vi "Test Format Entry Row.vi"(8 "error in":errorcluster, 10 "Work Folder":path, 11 "Test Data Folder":path) -> (0 "error out":errorcluster, 2 "Report":string, 3 "Passed":bool)   [LabVIEW 2026]
doc: "Tests Format Entry Row.vi with the Project Store of the schema-v2 sample data (Test Data\\Samples, copied into a new case folder). Checks: a row has the seven columns of the old TimeCard row (ID, Start, End, Elapsed, Project, Task, Description); an elapsed time of 59.6 s shows 00:01:00 and not 00:00:60; project and task names are looked up by ID; the Start column is the local time formatted %I:%M:%S %p; a running entry (End Time 0) gets an empty End column and an Elapsed of Now minus Start; an unknown Project ID is shown as the ID.\n\nInputs: Test Data Folder; Work Folder; error in. Outputs: Passed; Report; error out.\n\nGenerated by: Claude"
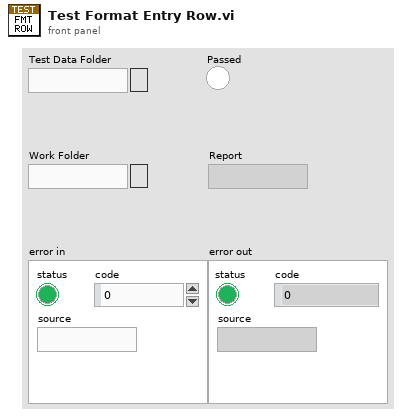
[diagram p1: front panel]
types:
  T1 = cluster{"ID":string, "Project ID":string, "Task ID":string, timestamp, timestamp, "Description":string}
  T2 = cluster{"ID":string, "Project ID":string, "Task ID":string, timestamp, "zero time":timestamp, "Description":string}
  T3 = cluster{"ID":string, "unknown project":string, "Task ID":string, timestamp, timestamp, "Description":string}
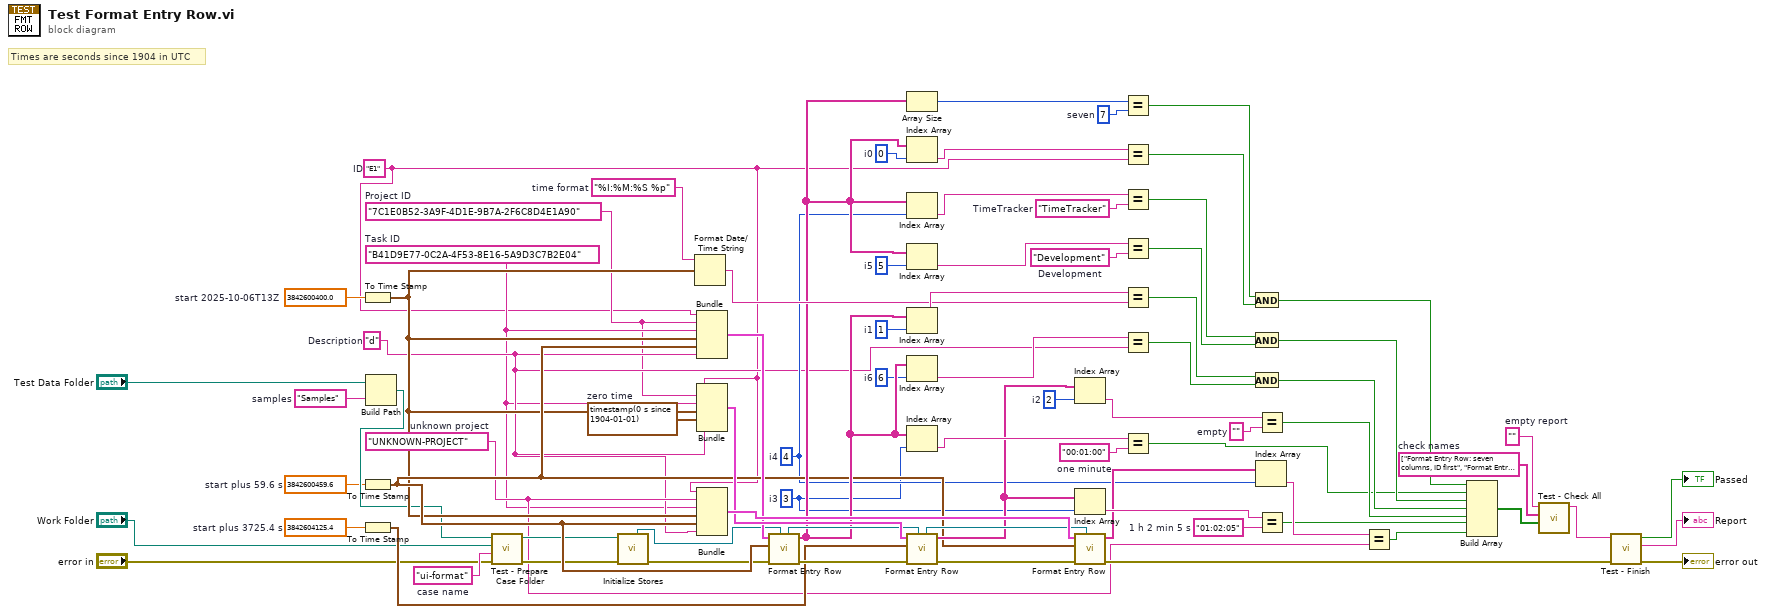
[diagram p0: block diagram]
diagram:
  w33 = string[] ["Format Entry Row: seven columns, ID first", "Format Entry Row: elapsed 59.6 s shows 00:01:00 (not 00:00:60)", "Format Entry Row: project and task names looked up by ID", "Format Entry Row: Start column is local %I:%M:%S %p and Description is last", "Format Entry Row: running entry leaves End empty", "Format Entry Row: running entry Elapsed is Now minus Start (01:02:05)", "Format Entry Row: unknown Project ID is shown as the ID"]  # check names
  w32 = "01:02:05"  # 1 h 2 min 5 s
  w31 = ""  # empty
  w30 = "Development"  # Development
  w29 = "TimeTracker"  # TimeTracker
  w28 = "00:01:00"  # one minute
  w27 = 6  # i6
  w26 = 5  # i5
  w25 = 4  # i4
  w24 = 3  # i3
  w23 = 2  # i2
  w22 = 1  # i1
  w21 = 0  # i0
  w20 = 7  # seven
  w19 = "%I:%M:%S %p"  # time format
  w18 = "UNKNOWN-PROJECT"  # unknown project
  w17 = timestamp(0 s since 1904-01-01)  # zero time
  w16 = 3842604125.4  # start plus 3725.4 s
  w15 = 3842600459.6  # start plus 59.6 s
  w14 = 3842600400.0  # start 2025-10-06T13Z
  w13 = "d"  # Description
  w12 = "B41D9E77-0C2A-4F53-8E16-5A9D3C7B2E04"  # Task ID
  w11 = "7C1E0B52-3A9F-4D1E-9B7A-2F6C8D4E1A90"  # Project ID
  w10 = "E1"  # ID
  w9 = ""  # empty report
  w8 = "ui-format"  # case name
  w7 = "Samples"  # samples
  # "Times are seconds since 1904 in UTC"
  n1 = To Time Stamp(1:w14) -> (0:w39:timestamp)
  n2 = To Time Stamp(1:w15) -> (0:w40:timestamp)
  n3 = To Time Stamp(1:w16) -> (0:w41:timestamp)
  n4 = Build Path(base path="Test Data Folder", name or relative path=w7) -> (appended path=w34:path)
  n5 = call "Test - Prepare Case Folder.vi"("error in (no error)"="error in", "Case Name"=w8, "Work Folder"="Work Folder", "Source Folder"=w34) -> ("error out"=w36:errorcluster, "Case Folder"=w35:path)  [unwired: 6 in]
  n6 = call "Initialize Stores.vi"("error in"=w36, "Data Folder"=w35) -> ("error out"=w38:errorcluster, "Project Store out"=w37:refnum<class "Project Store.lvclass">)  [unwired: 5 in, 3 out]
  n7 = Format Date/Time String(time format string (%c)=w19, seconds (now)=w39) -> (date/time string=w65:string)  [unwired: 1 out]
  n8 = Bundle("ID"=w10, "Project ID"=w11, "Task ID"=w12, w39, w40, "Description"=w13) -> (w42:T1)  [unwired: 1 in]
  n9 = Bundle("ID"=w10, "Project ID"=w11, "Task ID"=w12, w39, "zero time"=w17, "Description"=w13) -> (w46:T2)  [unwired: 1 in]
  n10 = Bundle("ID"=w10, "unknown project"=w18, "Task ID"=w12, w39, w40, "Description"=w13) -> (w50:T3)  [unwired: 1 in]
  n11 = call "Format Entry Row.vi"("Project Store in"=w37, "error in"=w38, "Now"=w40, "Time Entry"=w42) -> ("error out"=w45:errorcluster, "Row"=w43:string[], "Project Store out"=w44:refnum<class "Project Store.lvclass">)  [unwired: 5 in]
  n12 = Array Size(array=w43) -> (size(s)=w53:i32)
  n13 = Index Array(array=w43, index=w21) -> (element=w55:string)
  n14 = Index Array(array=w43, index=w25) -> (element=w60:string)
  n15 = Index Array(array=w43, index=w26) -> (element=w61:string)
  n16 = Index Array(array=w43, index=w22) -> (element=w66:string)
  n17 = Index Array(array=w43, index=w27) -> (element=w68:string)
  n18 = Index Array(array=w43, index=w24) -> (element=w58:string)
  n19 = call "Format Entry Row.vi"("Project Store in"=w44, "error in"=w45, "Now"=w41, "Time Entry"=w46) -> ("error out"=w49:errorcluster, "Row"=w47:string[], "Project Store out"=w48:refnum<class "Project Store.lvclass">)  [unwired: 5 in]
  n20 = Index Array(array=w47, index=w23) -> (element=w71:string)
  n21 = Index Array(array=w47, index=w24) -> (element=w73:string)
  n22 = call "Format Entry Row.vi"("Project Store in"=w48, "error in"=w49, "Now"=w40, "Time Entry"=w50) -> ("error out"=w52:errorcluster, "Row"=w51:string[])  [unwired: 5 in, 1 out]
  n23 = Equal?(x=w53, y=w20) -> (x = y?=w54:bool)
  n24 = Equal?(x=w55, y=w10) -> (x = y?=w56:bool)
  n25 = Equal?(x=w60, y=w29) -> (x = y?=w62:bool)
  n26 = Equal?(x=w61, y=w30) -> (x = y?=w63:bool)
  n27 = Equal?(x=w66, y=w65) -> (x = y?=w67:bool)
  n28 = Equal?(x=w68, y=w13) -> (x = y?=w69:bool)
  n29 = Equal?(x=w58, y=w28) -> (x = y?=w59:bool)
  n30 = And(x=w54, y=w56) -> (x .and. y?=w57:bool)
  n31 = And(x=w62, y=w63) -> (x .and. y?=w64:bool)
  n32 = And(x=w67, y=w69) -> (x .and. y?=w70:bool)
  n33 = Index Array(array=w51, index=w25) -> (element=w75:string)
  n34 = Equal?(x=w71, y=w31) -> (x = y?=w72:bool)
  n35 = Equal?(x=w73, y=w32) -> (x = y?=w74:bool)
  n36 = Equal?(x=w75, y=w18) -> (x = y?=w76:bool)
  n37 = Build Array(w57, w59, w64, w70, w72, w74, w76) -> (w77:bool[])
  n38 = call "Test - Check All.vi"("Conditions"=w77, "Check Names"=w33, "Report in"=w9) -> ("Report out"=w78:string)  [unwired: 7 in, 1 out]
  n39 = call "Test - Finish.vi"("error in (no error)"=w52, "Report"=w78) -> ("error out"=→"error out":errorcluster, "Report out"=→"Report":string, "Passed"=→"Passed":bool)  [unwired: 7 in]
